vi "Rev Set Encoder.vi"() -> ()   [LabVIEW 2027]
uses:
  <vilib>/REVLibDriver/REVLibDriver.lvlib
  <resource>/objmgr/REVSpark.rc
panel:
  out "error out 2":errorcluster
  out "error out":errorcluster
  out "after":sgl
  in  "EncoderPositionValue":sgl
  out "before":sgl
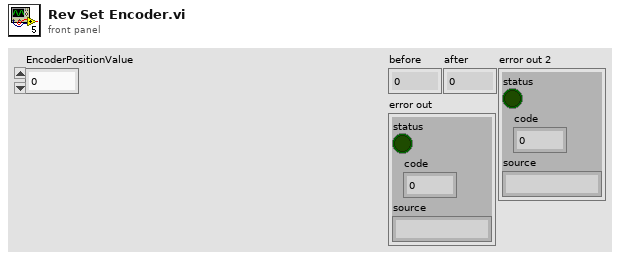
[diagram p1: front panel]
types:
  T1 = typedef "REVLibDriver.lvlib/REVSparkRefnum.ctl" = refnum<k20>
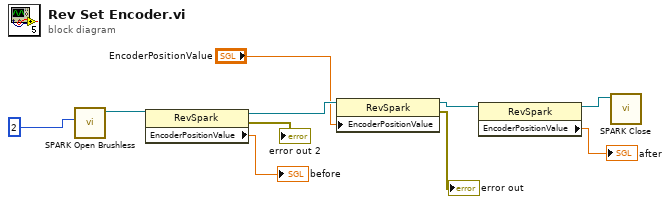
[diagram p0: block diagram]
diagram:
  n1 = call <vilib>:"SPARK Open Brushless.vi"("deviceId"=2) -> ("Spark refnum"=w9:T1)  [unwired: 9 in, 1 out]
  n2 = property class="RevSpark"(reference=w9) -> (reference out=w7:T1, error out=→"error out 2":errorcluster, "EncoderPositionValue"=→"before":sgl)  [unwired: 1 in]
  n3 = property class="RevSpark"(reference=w7, "EncoderPositionValue"="EncoderPositionValue") -> (reference out=w5:T1, error out=→"error out":errorcluster)  [unwired: 1 in]
  n4 = property class="RevSpark"(reference=w5) -> (reference out=w3:T1, "EncoderPositionValue"=→"after":sgl)  [unwired: 1 in, 1 out]
  n5 = call <vilib>:"SPARK Close.vi"("Spark refnum"=w3) -> ()  [unwired: 10 in, 1 out]
